vi "03 - Simple HTTP Data Connection.vi"() -> ()   [LabVIEW 2025]
uses:
  7801d39f-66b7-4e88-ad6f-c875adc63ad7.vi
  <vilib>/JDP Science/JSONtext/JSON text to Variant.vi
  <vilib>/JDP Science/JSONtext/LVClass Serializer/JSONtext LVClass Serializer.lvclass
  <vilib>/httpClient/LabVIEWHTTPClient.lvlib
panel:
  out "Element [0] Body":string
  in  "Stop":bool
  out "userId data":T1(array[cluster])
  out "raw JSON":string
  in  "user Id":i32=1
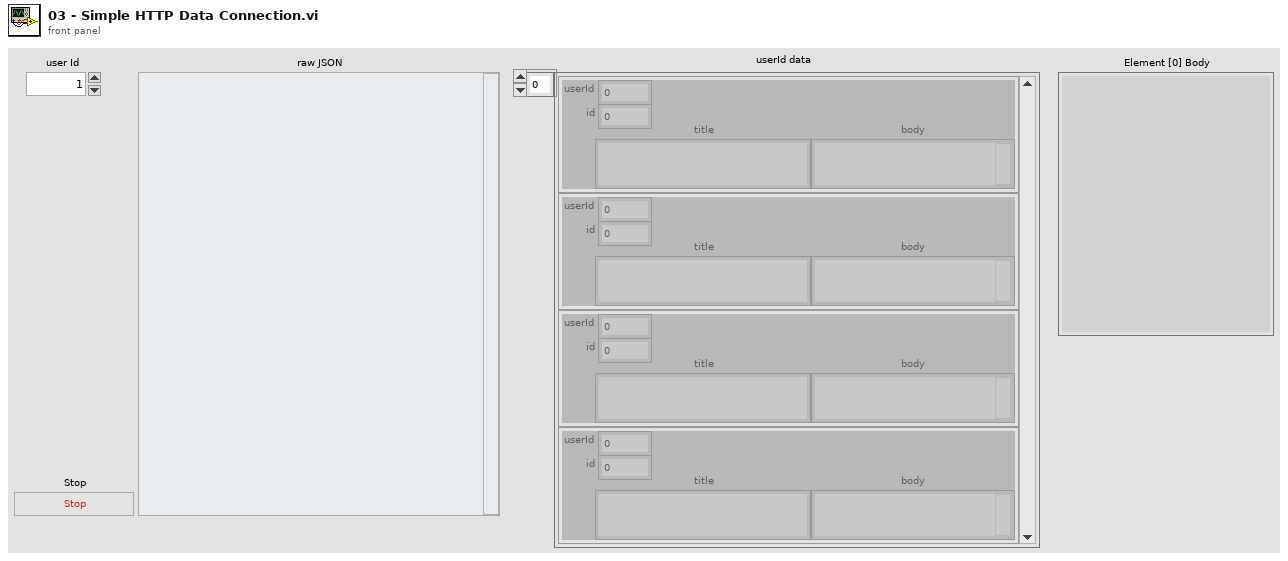
[diagram p1: front panel]
types:
  T1 = cluster{"userId":dbl, "id":dbl, "title":string, "body":string}[]
  T2 = typedef "LabVIEWHTTPClient.lvlib/ClientHandle.ctl" = refnum<k1>
  T3 = cluster{"userId":dbl, "id":dbl, "title":string, "body":string}
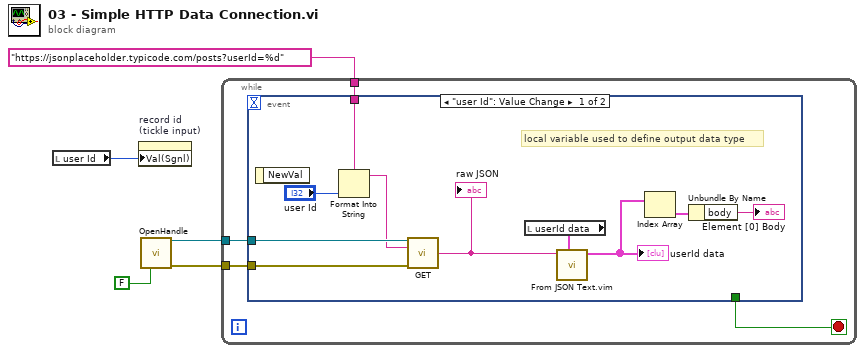
[diagram p0: block diagram]
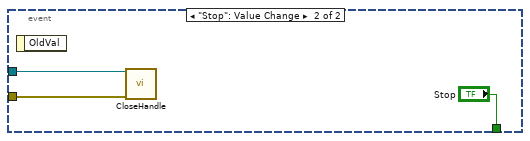
[diagram p2: hidden frame]
diagram:
  n1 = local read "user Id"() -> (w2:i32)
  n2 = property on="record id\n(tickle input)" class="DigNum (strict)"("Val(Sgnl)"=w2) -> ()  [unwired: 2 in, 2 out]
  n3 = call <vilib>:"OpenHandle.vi"("verify server(true)"=FALSE ("verify server (T)")) -> ("client handle out"=w3:T2, "error out"=w5:errorcluster)  [unwired: 13 in]
  n4 = while {
    tunnel: w3 -> [w8]
    tunnel: w5 -> [w9]
    tunnel: "https://jsonplaceholder.typicode.com/posts?userId=%d" ("url") -> [w7]
    stop <- w6 stop-if-true
    n5 = event shown="[0] \"user Id\": Value Change" {
      selector: _ -> [_ _]
      dyn-events: _ -> [_ _]
      timeout: _ -> [_ _]
      tunnel: w8 -> [w18 w20]
      tunnel: w9 -> [w19 w21]
      tunnel: w7 -> [w13 _]
      tunnel: [_ "Stop"] -> w6
      event "user Id": Value Change {
        # "local variable used to define output data type"
        n6 = event-data() -> ()  [unwired: 1 in, 1 out]
        n7 = Format Into String(format string=w13, "user Id") -> (resulting string=w17:string)  [unwired: 2 in, 1 out]
        n8 = call <vilib>:"GET.vi"("client handle"=w18, "url"=w17, "error in (no error)"=w19) -> ("body"=w15:string)  [unwired: 9 in, 3 out]
        "raw JSON" <- w15
        n9 = local read "userId data"() -> (w14:T1)
        n10 = call "From JSON Text.vim"("Data Type and Default Value"=w14, "JSON"=w15) -> ("Data out"=w12:T1)  [unwired: 8 in, 1 out]
        "userId data" <- w12
        n11 = Index Array(array=w12) -> (element=w11:T3)  [unwired: 1 in]
        n12 = Unbundle By Name(w11) -> ("body"=→"Element [0] Body":string)
      }
      event "Stop": Value Change {
        n13 = event-data() -> ()  [unwired: 1 in, 1 out]
        n14 = call <vilib>:"CloseHandle.vi"("client handle"=w20, "error in (no error)"=w21) -> ()  [unwired: 13 in, 1 out]
      }
    }
  }
